vi "Save Wfms.vi"(4 "Data File":T1, 8 "error in (no error)":errorcluster, 9 "V13_Wfm 2":waveform(dbl)={"t0"=timestamp(3404415606.9661703 s since 1904-01-01), "dt"=1.0299999999999546e-06, "Y"=array[1600 elements], "attributes"=variant("NI_ChannelName"=variant(string "Voltage"), "NI_UnitDescription"=variant(string "Volts"))}, 10 "V12_Wfm 2":waveform(dbl)={"t0"=timestamp(3404415606.9661703 s since 1904-01-01), "dt"=1.0299999999999546e-06, "Y"=array[1600 elements], "attributes"=variant("NI_ChannelName"=variant(string "Voltage"), "NI_UnitDescription"=variant(string "Volts"))}, 11 "V1 _Wfm":waveform(dbl)={"t0"=timestamp(3404415606.9661703 s since 1904-01-01), "dt"=1.0299999999999546e-06, "Y"=array[1600 elements], "attributes"=variant("NI_ChannelName"=variant(string "Voltage"), "NI_UnitDescription"=variant(string "Volts"))}) -> (0 "error out":errorcluster, 2 "Wfm":waveform(dbl)={"t0"=timestamp(3404415606.9661703 s since 1904-01-01), "dt"=1.0299999999999546e-06, "Y"=array[1600 elements], "attributes"=variant("NI_ChannelName"=variant(string "Voltage"), "NI_UnitDescription"=variant(string "Volts"))})   [LabVIEW 2013]
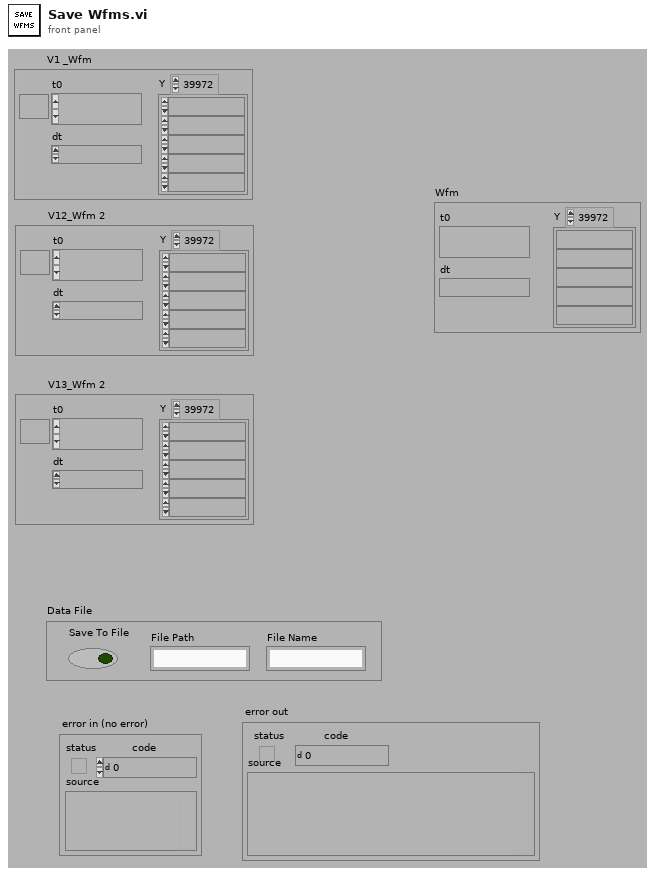
[diagram p1: front panel]
types:
  T1 = cluster{"File Name":string, "File Path":string, "Save To File":bool}
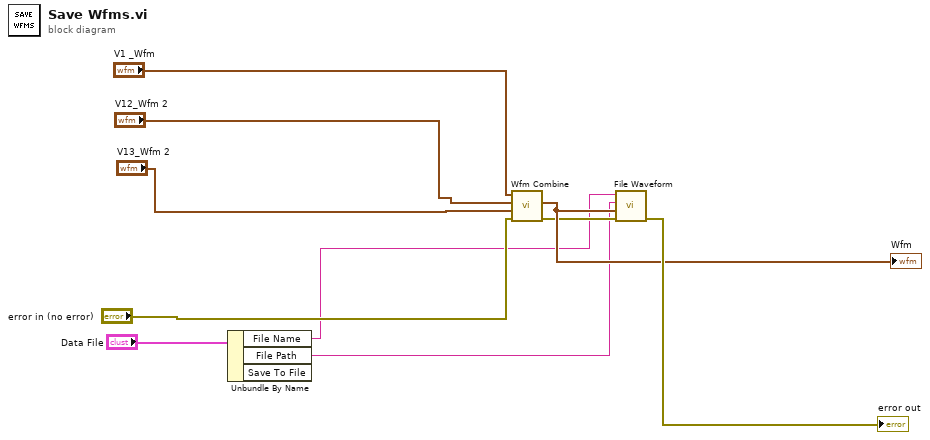
[diagram p0: block diagram]
diagram:
  n1 = Unbundle By Name("Data File") -> ("File Name"=w5:string, "File Path"=w4:string)  [unwired: 1 out]
  n2 = call "Wfm Combine.vi"("error in (no error)"="error in (no error)", "Wfm3"="V13_Wfm 2", "Wfm2"="V12_Wfm 2", "Wfm1"="V1 _Wfm") -> ("error out"=w6:errorcluster, "Output Wfm"=w8:waveform(dbl))  [unwired: 6 in]
  "Wfm" <- w8
  n3 = call "File Waveform.vi"("error in (no error)"=w6, "waveform"=w8, "File Path"=w4, "File Name"=w5) -> ("error out"=→"error out":errorcluster)  [unwired: 5 in, 2 out]
